vi "Read_Full.vi"(7 "CheckFaults":bool, 8 "error in (no error)":errorcluster, 9 "Results Array In":dbl[](array[numeric]), 11 "SoftmotionAxis in":refnum<class "SoftmotionAxis.lvclass">) -> (0 "error out":errorcluster, 1 "appended array":dbl[](array[numeric]), 3 "SoftmotionAxis out":refnum<class "SoftmotionAxis.lvclass">)   [LabVIEW 2017, in "SoftmotionAxis.lvclass"]
uses:
  SoftmotionAxis.lvclass
  <resource>/objmgr/nimcai.rc
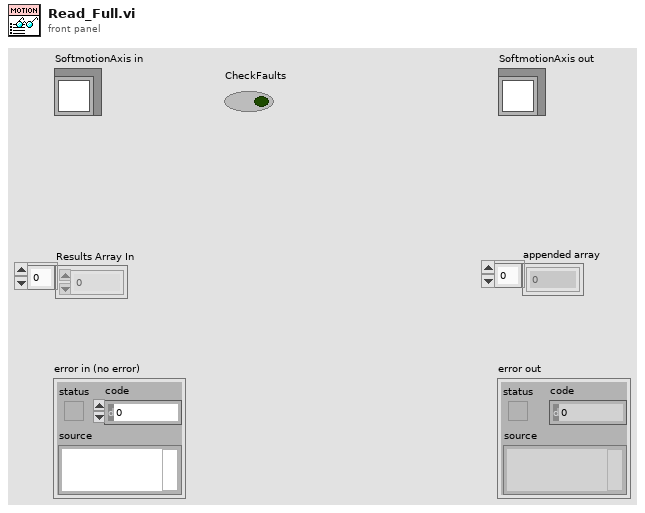
[diagram p1: front panel]
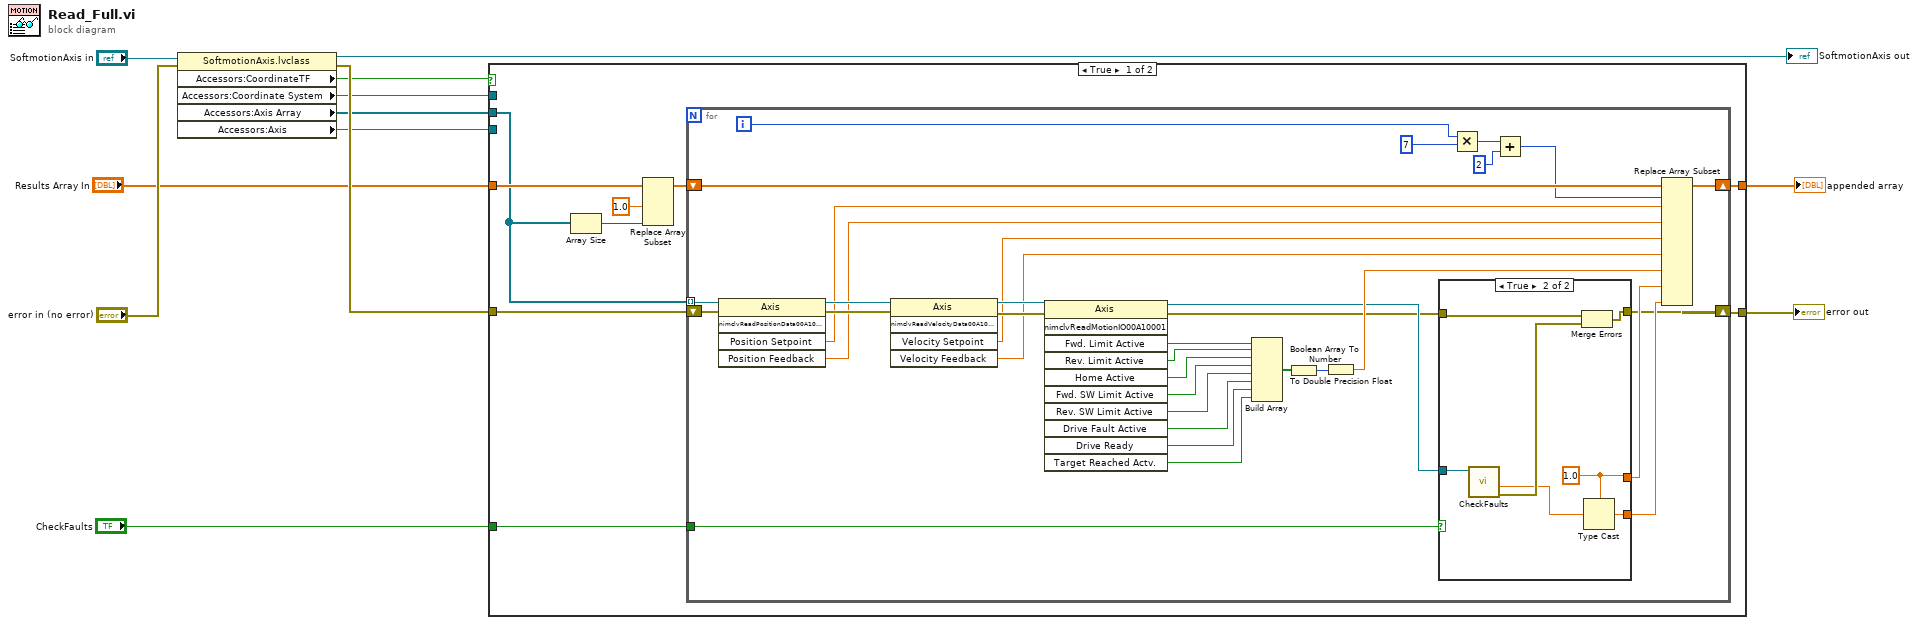
[diagram p0: block diagram]
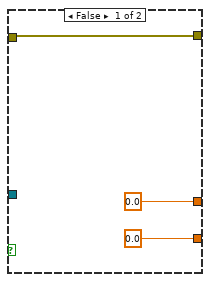
[diagram p2: hidden frame]
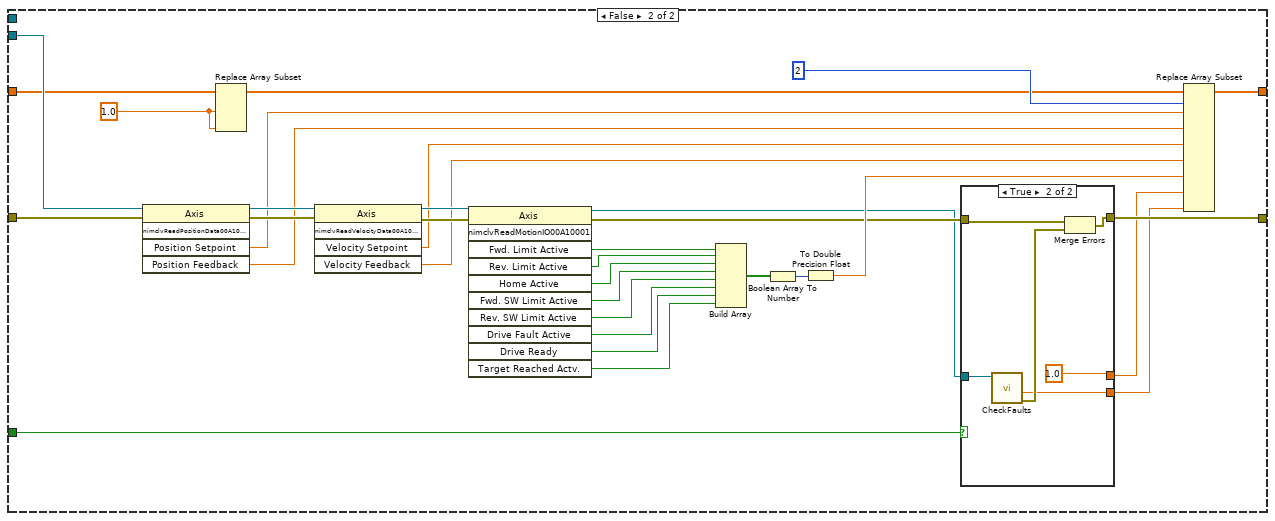
[diagram p3: hidden frame]
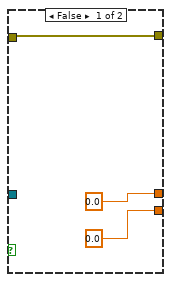
[diagram p4: hidden frame]
diagram:
  n1 = property class="SoftmotionAxis.lvclass"(reference="SoftmotionAxis in", error in="error in (no error)") -> (reference out=→"SoftmotionAxis out":refnum<class "SoftmotionAxis.lvclass">, error out=w12:errorcluster, "Accessors:CoordinateTF"=w10:bool, "Accessors:Coordinate System"=w9:refnum<k21>, "Accessors:Axis Array"=w3:refnum<k21>[], "Accessors:Axis"=w11:refnum<k21>)
  n2 = case shown="True" w10 {
    tunnel: [w19 w81] -> w6
    tunnel: [w21 w70] -> w5
    tunnel: w12 -> [w20 w87]
    tunnel: w11 -> [_ w82]
    tunnel: w9 -> [_ _]
    tunnel: w3 -> [w15 _]
    tunnel: "Results Array In" -> [w17 w74]
    tunnel: "CheckFaults" -> [w13 w69]
    frame True {
      n3 = Array Size(array=w15) -> (size(s)=w14:i32)
      n4 = Replace Array Subset(array=w17, new element #1=1.0 ("new element/subarray"), new element #2=w14) -> (w16:dbl[])  [unwired: 2 in]
      n5 = for {
        shift-right: [w25] -> w21
        shift-left: w20 -> [w46]
        tunnel: w15 -> [w41] mode=indexing
        shift-right: [w36] -> w19
        shift-left: w16 -> [w35]
        tunnel: w13 -> [w29]
        i -> [w40]
        n6 = invoke class="Axis" method="nimclvReadPositionData00A10001"(reference=w41, error in=w46) -> (reference out=w45:refnum<k21>, error out=w44:errorcluster, "Position Setpoint"=w38:dbl, "Position Feedback"=w37:dbl)  [unwired: 3 in, 1 out]
        n7 = invoke class="Axis" method="nimclvReadVelocityData00A10001"(reference=w45, error in=w44) -> (reference out=w43:refnum<k21>, error out=w42:errorcluster, "Velocity Setpoint"=w34:dbl, "Velocity Feedback"=w33:dbl)  [unwired: 3 in, 1 out]
        n8 = invoke class="Axis" method="nimclvReadMotionIO00A10001"(reference=w43, error in=w42) -> (reference out=w27:refnum<k21>, error out=w26:errorcluster, "Fwd. Limit Active"=w55:bool, "Rev. Limit Active"=w54:bool, "Home Active"=w53:bool, "Fwd. SW Limit Active"=w52:bool, "Rev. SW Limit Active"=w51:bool, "Drive Fault Active"=w50:bool, "Drive Ready"=w49:bool, "Target Reached Actv."=w28:bool)  [unwired: 9 in, 1 out]
        n9 = Build Array(w55, w54, w53, w52, w51, w50, w49, w28) -> (w48:bool[])
        n10 = Boolean Array To Number(Boolean array=w48) -> (number=w47:u32)
        n11 = To Double Precision Float(number=w47) -> (double precision float=w32:dbl)
        n12 = case shown="True" w29 {
          tunnel: [0.0 ("y") w61] -> w31
          tunnel: [0.0 ("y") w60] -> w30
          tunnel: w27 -> [_ w65]
          tunnel: w26 -> [w56 w64]
          tunnel: [w56 w62] -> w25
          frame False {
          }
          frame True {
            w61 = 1.0 ("y")
            n13 = call "CheckFaults.vi"("Axis"=w65) -> ("error out"=w63:errorcluster, "Numeric"=w59:dbl)  [unwired: 9 in]
            n14 = Merge Errors(w64, w63) -> (w62:errorcluster)
            n15 = Type Cast(type=w61, x=w59) -> (*(type *) &x=w60:dbl)
          }
        }
        n16 = Multiply(x=w40, y=7) -> (x*y=w24:i32)
        n17 = Add(x=w24, y=2) -> (x+y=w22:i32)
        n18 = Replace Array Subset(array=w35, new element #1=w38, index #1=w22, new element #2=w37, new element #3=w34, new element #4=w33, new element #5=w32, new element #6=w31, new element #7=w30) -> (w36:dbl[])  [unwired: 6 in]
      }
    }
    frame False {
      w72 = 1.0 ("new element/subarray")
      n19 = invoke class="Axis" method="nimclvReadPositionData00A10001"(reference=w82, error in=w87) -> (reference out=w86:refnum<k21>, error out=w85:errorcluster, "Position Setpoint"=w79:dbl, "Position Feedback"=w80:dbl)  [unwired: 3 in, 1 out]
      n20 = Replace Array Subset(array=w74, new element #1=w72, new element #2=w72) -> (w73:dbl[])  [unwired: 2 in]
      n21 = invoke class="Axis" method="nimclvReadVelocityData00A10001"(reference=w86, error in=w85) -> (reference out=w84:refnum<k21>, error out=w83:errorcluster, "Velocity Setpoint"=w76:dbl, "Velocity Feedback"=w77:dbl)  [unwired: 3 in, 1 out]
      n22 = invoke class="Axis" method="nimclvReadMotionIO00A10001"(reference=w84, error in=w83) -> (reference out=w68:refnum<k21>, error out=w71:errorcluster, "Fwd. Limit Active"=w97:bool, "Rev. Limit Active"=w96:bool, "Home Active"=w95:bool, "Fwd. SW Limit Active"=w94:bool, "Rev. SW Limit Active"=w93:bool, "Drive Fault Active"=w92:bool, "Drive Ready"=w91:bool, "Target Reached Actv."=w90:bool)  [unwired: 9 in, 1 out]
      n23 = Build Array(w97, w96, w95, w94, w93, w92, w91, w90) -> (w89:bool[])
      n24 = Boolean Array To Number(Boolean array=w89) -> (number=w88:u32)
      n25 = To Double Precision Float(number=w88) -> (double precision float=w78:dbl)
      n26 = case shown="True" w69 {
        tunnel: [0.0 ("y") 1.0 ("y")] -> w67
        tunnel: [0.0 ("y") w101] -> w66
        tunnel: w68 -> [_ w106]
        tunnel: w71 -> [w98 w105]
        tunnel: [w98 w103] -> w70
        frame False {
        }
        frame True {
          n27 = call "CheckFaults.vi"("Axis"=w106) -> ("error out"=w104:errorcluster, "Numeric"=w101:dbl)  [unwired: 9 in]
          n28 = Merge Errors(w105, w104) -> (w103:errorcluster)
        }
      }
      n29 = Replace Array Subset(array=w73, new element #1=w79, index #1=2 ("index"), new element #2=w80, new element #3=w76, new element #4=w77, new element #5=w78, new element #6=w67, new element #7=w66) -> (w81:dbl[])  [unwired: 6 in]
    }
  }
  "error out" <- w5
  "appended array" <- w6
